vi "Analog_Write.vi"(8 "error in (no error)":errorcluster, 9 "Valor":u8, 10 "Canal":u8, 11 "VISA resource name":refnum<visa-resource-name>) -> (0 "error out":errorcluster, 3 "VISA resource name out":refnum<visa-resource-name>)   [LabVIEW 2026]
panel:
  out "respuesta":string
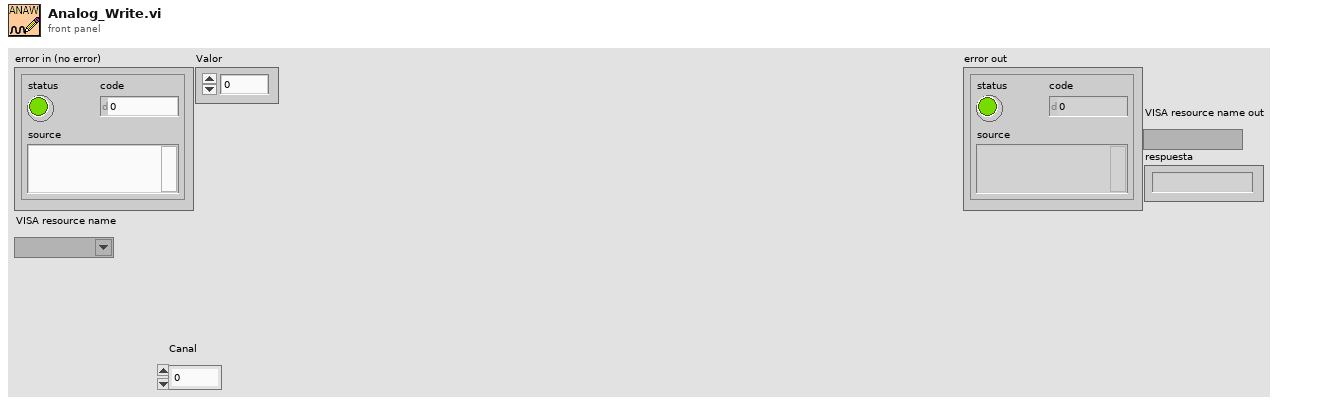
[diagram p1: front panel]
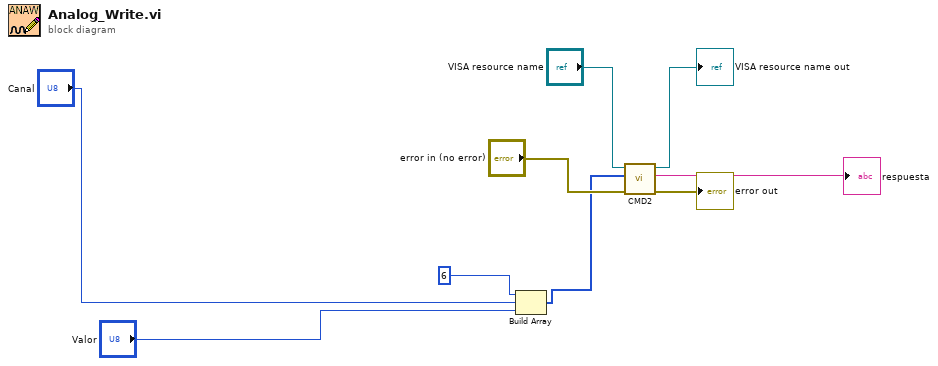
[diagram p0: block diagram]
diagram:
  n1 = Build Array(u8 6, "Canal", "Valor") -> (w3:u8[])
  n2 = call "CMD2.vi"("error in (no error)"="error in (no error)", "Comando"=w3, "VISA resource name"="VISA resource name") -> ("error out"=→"error out":errorcluster, "respuesta"=→"respuesta":string, "VISA resource name out"=→"VISA resource name out":refnum<visa-resource-name>)  [unwired: 6 in]
